vi "ASK Modulator.vi"() -> ()   [LabVIEW 2026]
panel:
  out "ASK Waveform":dbl[](graph)
  out "ASK Modulated Signal":dbl[](array[numeric])
  in  "Carrier Amplitude(A)":dbl
  in  "Carrier Frequency(fc)":dbl
  in  "Sampling Frequency(Fs)":dbl
  in  "Baseband Signal":dbl[](array[numeric])
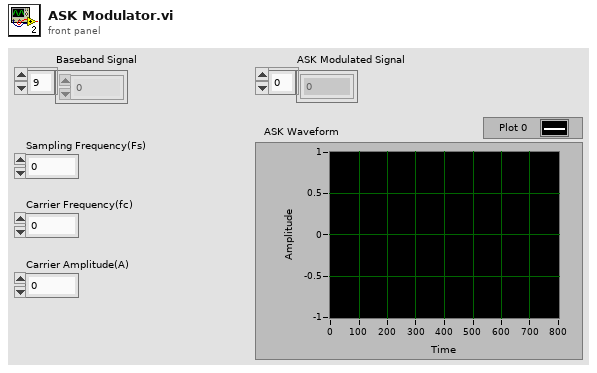
[diagram p1: front panel]
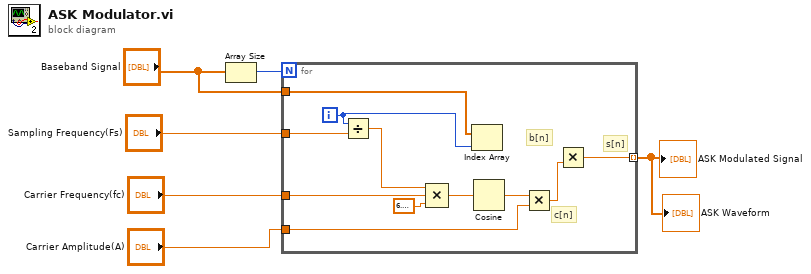
[diagram p0: block diagram]
diagram:
  n1 = Array Size(array="Baseband Signal") -> (size(s)=w6:i32)
  n2 = for {
    N: w6 -> [_]
    tunnel: "Sampling Frequency(Fs)" -> [w17]
    tunnel: "Carrier Frequency(fc)" -> [w15]
    tunnel: "Carrier Amplitude(A)" -> [w11]
    tunnel: [w8] -> w3 mode=indexing
    tunnel: "Baseband Signal" -> [w7]
    i -> [w10]
    # "s[n]"
    # "c[n]"
    # "b[n]"
    n3 = Divide(x=w10, y=w17) -> (x/y=w16:dbl)
    n4 = Compound Arithmetic op=MULTIPLY(w16, w15, 6.283185307179586) -> (w13:dbl)
    n5 = Index Array(array=w7, index=w10) -> ()  [unwired: 1 out]
    n6 = Cosine(x=w13) -> (cos(x)=w12:dbl)
    n7 = Multiply(x=w12, y=w11) -> (x*y=w9:dbl)
    n8 = Multiply(y=w9) -> (x*y=w8:dbl)  [unwired: 1 in]
  }
  "ASK Modulated Signal" <- w3
  "ASK Waveform" <- w3
